vi "ZM-ROOT-close.vi"(8 "error in (no error)":errorcluster, 11 "ZM-ROOT-root in":refnum<class "ZM-ROOT-root.lvclass">) -> (0 "error out":errorcluster, 3 "ZM-ROOT-root out":refnum<class "ZM-ROOT-root.lvclass">)   [LabVIEW 2020, in "ZM-ROOT-root.lvlib" / "ZM-ROOT-root.lvclass"]
doc: "Destroys the root's stop and error user events, called at the end of Actor Core and after a failed create. Release errors (an event never created) are ignored; error in passes through."
uses:
  ZM-ROOT-root.lvclass
  ZM-ROOT-root.lvclass/ZM-ROOT-root.ctl
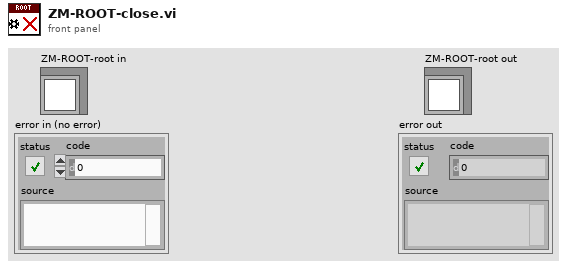
[diagram p1: front panel]
types:
  T1 = typedef "ZM-ROOT-root.lvlib/ZM-ROOT-root.lvclass/ZM-ROOT-EVENTS.ctl" = cluster{"stop":refnum<user-event>, "error":refnum<user-event>}
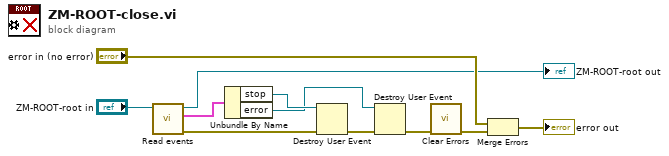
[diagram p0: block diagram]
diagram:
  n1 = call "Read events.vi"("ZM-ROOT-root in"="ZM-ROOT-root in") -> ("error out"=w8:errorcluster, "ZM-ROOT-EVENTS"=w10:T1, "ZM-ROOT-root out"=→"ZM-ROOT-root out":refnum<class "ZM-ROOT-root.lvclass">)  [unwired: 8 in]
  n2 = Unbundle By Name(w10) -> ("stop"=w9:refnum<user-event>, "error"=w7:refnum<user-event>)
  n3 = Destroy User Event(user event=w9, error in=w8) -> (error out=w6:errorcluster)
  n4 = Destroy User Event(user event=w7, error in=w6) -> (error out=w5:errorcluster)
  n5 = call <vilib>:"Clear Errors.vi"("error in (no error)"=w5) -> ("error out"=w3:errorcluster)  [unwired: 5 in, 1 out]
  n6 = Merge Errors("error in (no error)", w3) -> (→"error out":errorcluster)
